vi "PathPlanner_ObstacleGrid_ReadNavFile.vi"(11 "FileName":string="default_navgrid.json") -> (0 "error out":errorcluster, 2 "NavGridObstacles":T1[](array[typedef]), 3 "PathPlanner_Grid":T2, 4 "Full Filename":string)   [LabVIEW 2019, in "PathPlanner24.lvlib"]
doc: "Load an obstacle grid from a JSON formatted file. \n\nInputs: \n - filename - string - The name of the obstacle grid file. See notes below on file naming.\n\nOutputs:\n - PathPlanner_ObstacleGrid - cluster - Obstacle grid read from JSON file.\n - Error out - cluster - Error cluster\n - Full Filename - string - fully qualified file name.\n\nNotes on file naming:\n - The file name must include the extention. \".json\" is not automatically appended to the name. \n - The file name can be a simple file or an absolute path. If a simple file name is used the default path on the RoboRIO is: \"home:\\lvuser\\natinst\\LabVIEW Data\". On a Windows PC the default path is the LabVIEW default directory. Normally this is: “%HOMEDRIVE%%HOMEPATH%\\Documents\\LabView Data\".\n - Filenames on the RoboRIO, which runs Linux, are case sensitive.\ni"
uses:
  PathPlanner24.lvlib
  TypeDef/PathPlannerObstacleGrid.ctl
  TypeDef/PathPlannerFinderGridPosition.ctl
panel:
  in  "error in (no error)":errorcluster
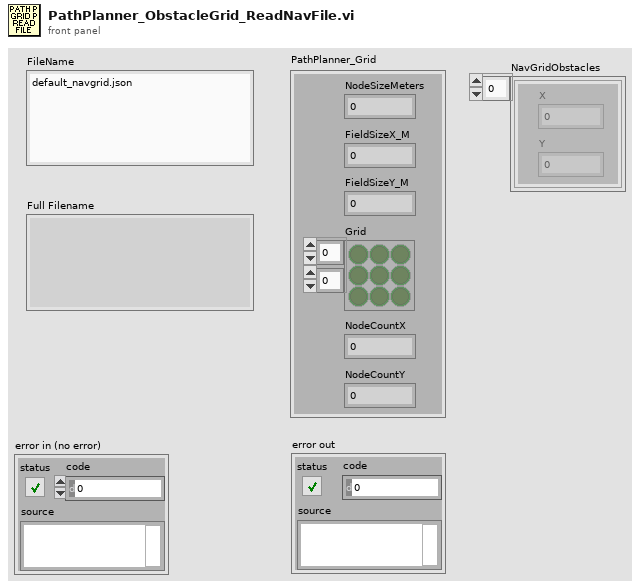
[diagram p1: front panel]
types:
  T1 = typedef "PathPlanner24.lvlib/PathPlannerFinderGridPosition.ctl" = cluster{"X":i32, "Y":i32}
  T2 = typedef "PathPlanner24.lvlib/PathPlannerObstacleGrid.ctl" = cluster{"NodeSizeMeters":dbl, "Grid":bool[][], "NodeCountX":i32, "NodeCountY":i32, "FieldSizeX_M":dbl, "FieldSizeY_M":dbl}
  T3 = enum16{"open", "replace", "create", "open or create", "replace or create", "replace or create with confirmation"}
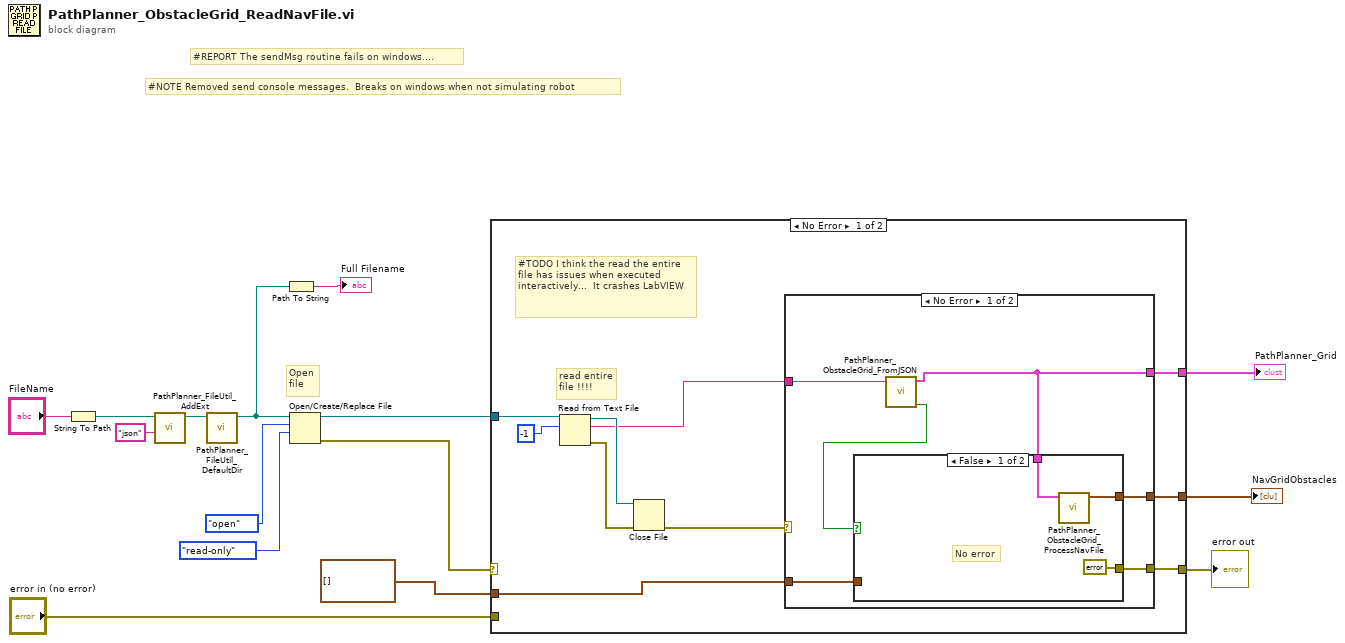
[diagram p0: block diagram]
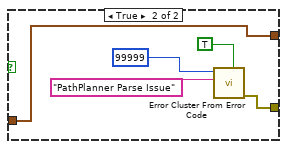
[diagram p2: hidden frame]
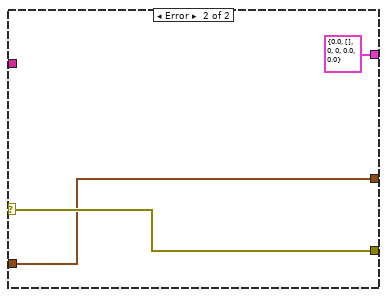
[diagram p3: hidden frame]
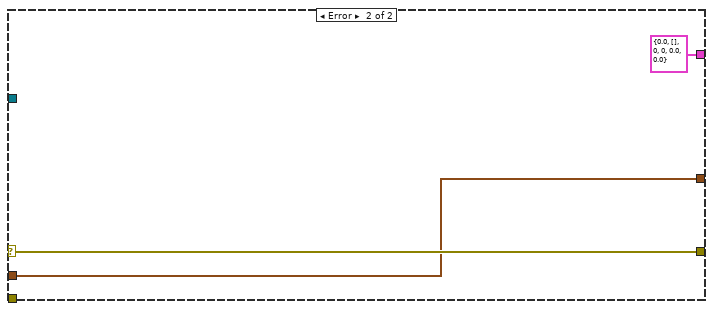
[diagram p4: hidden frame]
diagram:
  # "#NOTE Removed send console messages.  Breaks on windows when not simulating robot"
  # "#REPORT The sendMsg routine fails on windows...."
  # "Open\nfile"
  n1 = String To Path(string="FileName") -> (path=w4:path)
  n2 = call "PathPlanner_FileUtil_AddExt.vi"("Extension"="json", "Path in"=w4) -> ("Path out"=w2:path)  [unwired: 9 in]
  n3 = call "PathPlanner_FileUtil_DefaultDir.vi"("Path in"=w2) -> ("Path Out"=w1:path)  [unwired: 10 in]
  n4 = Path To String(path=w1) -> (string=→"Full Filename":string)
  n5 = Open/Create/Replace File(file path (use dialog)=w1, operation (0:open)=T3."open", access (0:read/write)=enum16{"read/write", "read-only", "write-only"}."read-only") -> (refnum out=w11:refnum<file>, error out=w13:errorcluster)  [unwired: 3 in, 1 out]
  n6 = case shown="No Error" w13 {
    selector: w13 -> [_ w45]
    tunnel: w11 -> [w24 _]
    tunnel: [w19 w45] -> w8
    tunnel: "error in (no error)" -> [_ _]
    tunnel: [w18 T2 {"NodeSizeMeters"=0.0, "Grid"=[], "NodeCountX"=0, "NodeCountY"=0, "FieldSizeX_M"=0.0, "FieldSizeY_M"=0.0} ("PathPlanner_Grid")] -> w7
    tunnel: [w17 w43] -> w6
    tunnel: T1[] [] ("NavGridObstacles") -> [w16 w43]
    frame No Error {
      # "#TODO I think the read the entire\nfile has issues when executed\ninteractively...  It crashes LabVIEW"
      # "read entire\nfile !!!!"
      n7 = Read from Text File(file (use dialog)=w24, count=-1) -> (refnum out=w23:refnum<file>, text=w22:string, error out=w21:errorcluster)  [unwired: 2 in, 1 out]
      n8 = Close File(refnum=w23, error in=w21) -> (error out=w20:errorcluster)  [unwired: 1 out]
      n9 = case shown="No Error" w20 {
        selector: w20 -> [_ w42]
        tunnel: w22 -> [w31 _]
        tunnel: [w29 w42] -> w19
        tunnel: [w28 T2 {"NodeSizeMeters"=0.0, "Grid"=[], "NodeCountX"=0, "NodeCountY"=0, "FieldSizeX_M"=0.0, "FieldSizeY_M"=0.0} ("PathPlanner_Grid")] -> w18
        tunnel: [w27 w40] -> w17
        tunnel: w16 -> [w26 w40]
        frame No Error {
          n10 = call "PathPlanner_ObstacleGrid_FromJSON.vi"("JSON String"=w31) -> ("Error"=w30:bool, "PathPlanner_Grid"=w28:T2)  [unwired: 9 in]
          n11 = case shown="False" w30 {
            tunnel: [errorcluster {"status"=FALSE, "code"=0, "source"=""} ("error out") w36] -> w29
            tunnel: w28 -> [w33 _]
            tunnel: [w32 w35] -> w27
            tunnel: w26 -> [_ w35]
            frame False {
              # "No error"
              n12 = call "PathPlanner_ObstacleGrid_ProcessNavFile.vi"("PathPlanner_Grid"=w33) -> ("NavGridObstacles"=w32:T1[])  [unwired: 10 in]
            }
            frame True {
              n13 = call <vilib>:"Error Cluster From Error Code.vi"("is warning? (False)"=TRUE, "error message (\"\")"="PathPlanner Parse Issue" ("error message (\"\")"), "error code (0)"=99999) -> ("error out"=w36:errorcluster)  [unwired: 6 in]
            }
          }
        }
        frame Error {
        }
      }
    }
    frame Error {
    }
  }
  "error out" <- w8
  "PathPlanner_Grid" <- w7
  "NavGridObstacles" <- w6
